vi "json_cluster.vi"(7 "indent level":i32, 10 "array of JSON values":string[](array[string]), 11 "array of element names":string[](array[string])) -> (3 "indented string":string)   [LabVIEW 2020, in "Caraya.lvlib" / "Test Result.lvclass"]
uses:
  Test Result.lvclass
  <vilib>/Utility/error.llb/whitespace.ctl
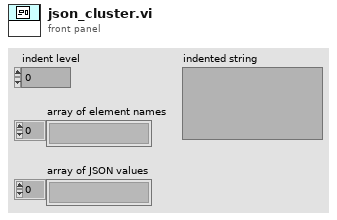
[diagram p1: front panel]
types:
  T1 = typedef "whitespace.ctl" = u16
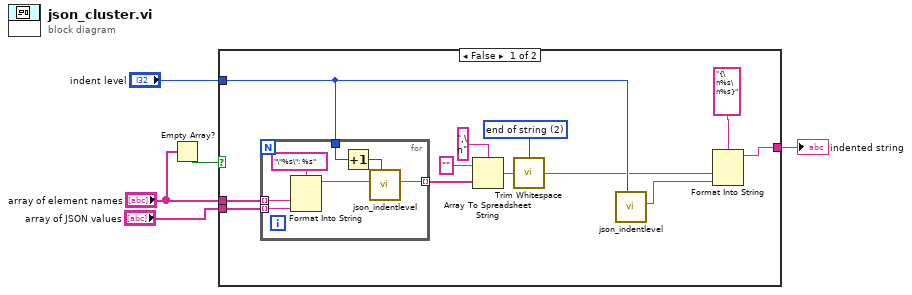
[diagram p0: block diagram]
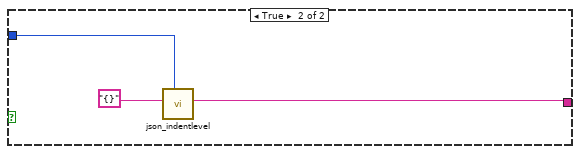
[diagram p2: hidden frame]
diagram:
  n1 = Empty Array?(array="array of element names") -> (empty?=w1:bool)
  n2 = case shown="False" w1 {
    tunnel: "indent level" -> [w17 w27]
    tunnel: "array of JSON values" -> [w10 _]
    tunnel: [w8 w25] -> w3
    tunnel: "array of element names" -> [w6 _]
    frame False {
      w13 = T1 2 items=["both", "start of string", "end of string"] ("location (both)")
      n3 = for {
        tunnel: w6 -> [w24] mode=indexing
        tunnel: w10 -> [w23] mode=indexing
        tunnel: [w20] -> w15 mode=indexing
        tunnel: w17 -> [w19]
        n4 = Format Into String(format string="\"%s\": %s" ("string"), w24, w23) -> (resulting string=w21:string)  [unwired: 2 in, 1 out]
        n5 = Increment(x=w19) -> (x+1=w18:i32)
        n6 = call "json_indentlevel.vi"("indent level"=w18, "string"=w21) -> ("indented string"=w20:string)  [unwired: 9 in]
      }
      n7 = Array To Spreadsheet String(delimiter (Tab)=",\n", array=w15, 3:"" ("format string")) -> (spreadsheet string=w14:string)
      n8 = call <vilib>:"Trim Whitespace.vi"("string"=w14, "location (both)"=w13) -> ("trimmed string"=w16:string)
      n9 = call "json_indentlevel.vi"("indent level"=w17) -> ("indented string"=w9:string)  [unwired: 10 in]
      n10 = Format Into String(format string="{\n%s\n%s}", w16, w9) -> (resulting string=w8:string)  [unwired: 2 in, 1 out]
    }
    frame True {
      n11 = call "json_indentlevel.vi"("indent level"=w27, "string"="{}") -> ("indented string"=w25:string)  [unwired: 9 in]
    }
  }
  "indented string" <- w3
